vi "ReadSensorMake.vi"(8 "Error In":errorcluster, 11 "object in":refnum<class "Controller.lvclass">) -> (0 "Error Out":errorcluster, 2 "SensorMake":T1, 3 "object out":refnum<class "Controller.lvclass">)   [LabVIEW 2022 SP3, in "Controller.lvlib" / "Controller.lvclass"]
uses:
  Controller.lvclass
  TypeDef/SensorMake.ctl
  Controller.lvclass/Controller.ctl
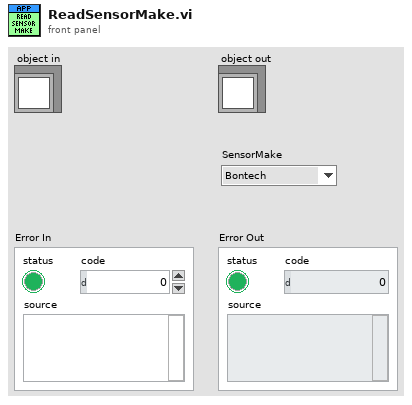
[diagram p1: front panel]
types:
  T1 = typedef "SensorMake.ctl" = enum16{"Bontech", "DTImaging", "VarexImaging"}
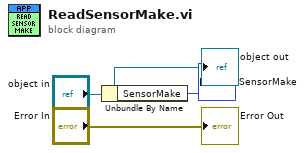
[diagram p0: block diagram]
diagram:
  n1 = Unbundle By Name("object in") -> ("SensorMake"=→"SensorMake":T1)
  "Error Out" <- "Error In"
  "object out" <- "object in"
